vi "RunTimeObjectsSectionUI.vi"() -> ()   [LabVIEW 2015, in "RunTimeObjectsSection.lvclass"]
uses:
  RunTimeObjectsSection.lvclass
  <vilib>/NI/Configuration Framework/Node/NodeRef.ctl
  <vilib>/NI/Configuration Framework/Node/NISE_CEF_Node.lvclass
  <vilib>/NI/AMC/Message Queue.ctl
  <vilib>/NI/AMC/Message.ctl
  <vilib>/NI/Tools/Keyed Array/KeyedArray.ctl
  <vilib>/NI/Configuration Framework/Node/UserEventRef.ctl
  <vilib>/NI/Configuration Framework/Controls/EventCluster.ctl
  <vilib>/Utility/sysdir.llb/System Directory Type.ctl
  Controls/RunTimeObjectTypes.ctl
  RunTimeObjectsSection.lvclass/RunTimeObjectsSection.ctl
  Read RunTimeObjectType.vi
  subVI/Global Settings.vi
  Configuration Tool.lvlib
  <vilib>/NI/Tools/Keyed Array/Tools_KeyedArray.lvlib
  <vilib>/NI/AMC/AMC.lvlib
  <vilib>/NI/Configuration Framework/NISE_CEF_TreeControl.lvlib
panel:
  in  "Main UI Tab":enum32{"Page Group"}(tab)
  in  "WebBrowser":refnum<k7>(container)
  in  "user event":T1
  in  "main queue":T2
  in  "node ref":T3
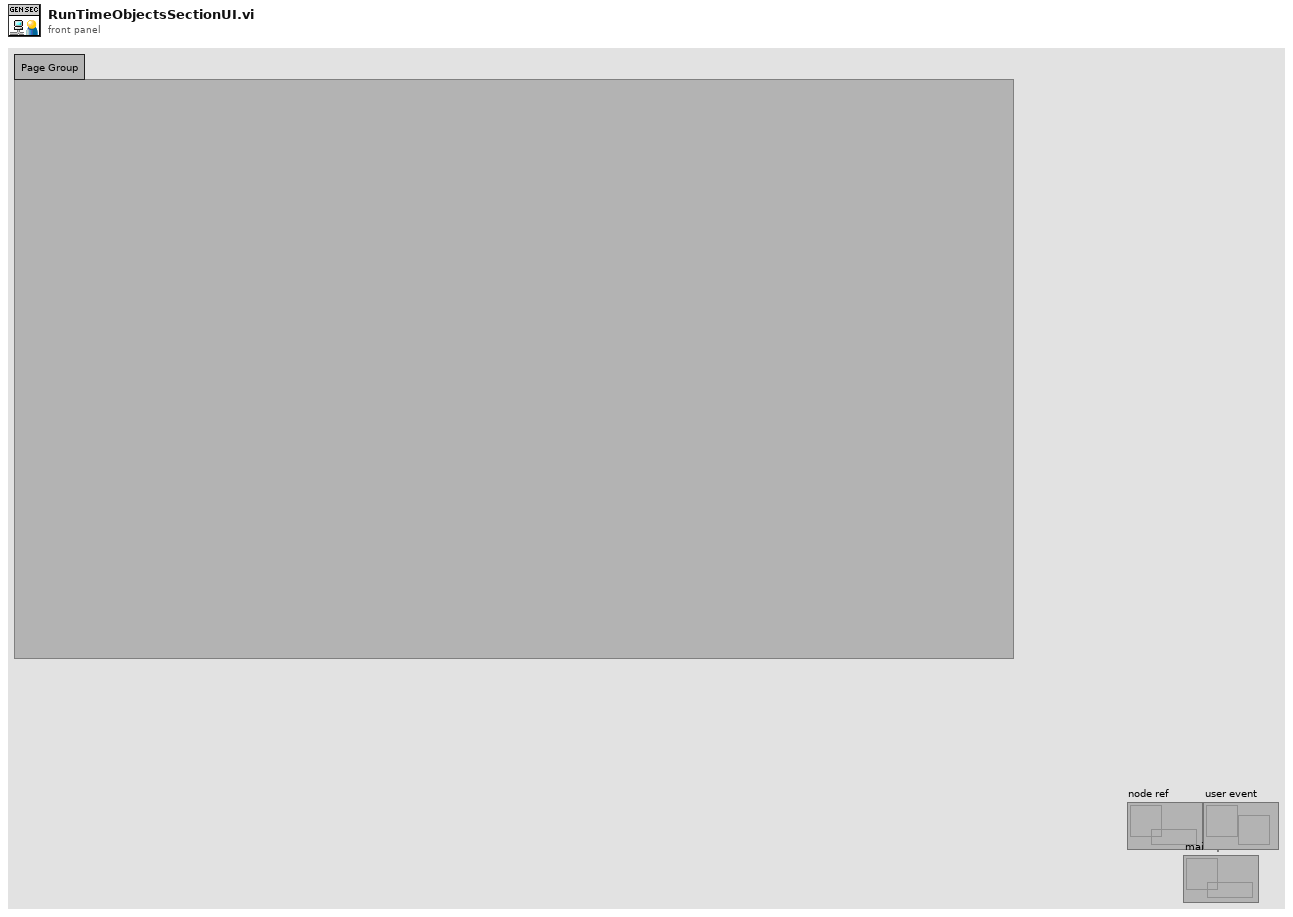
[diagram p1: front panel]
types:
  T1 = typedef "NISE_CEF_Node.lvclass/UserEventRef.ctl" = refnum<user-event>
  T2 = typedef "AMC.lvlib/Message Queue.ctl" = refnum<queue>
  T3 = typedef "NISE_CEF_Node.lvclass/NodeRef.ctl" = refnum<data-value>
  T4 = typedef "Configuration Tool.lvlib/RunTimeObjectTypes.ctl" = enum16{"ActionVIs", "ButtonList", "RunTimeMenu"}
  T5 = typedef "System Directory Type.ctl" = i32
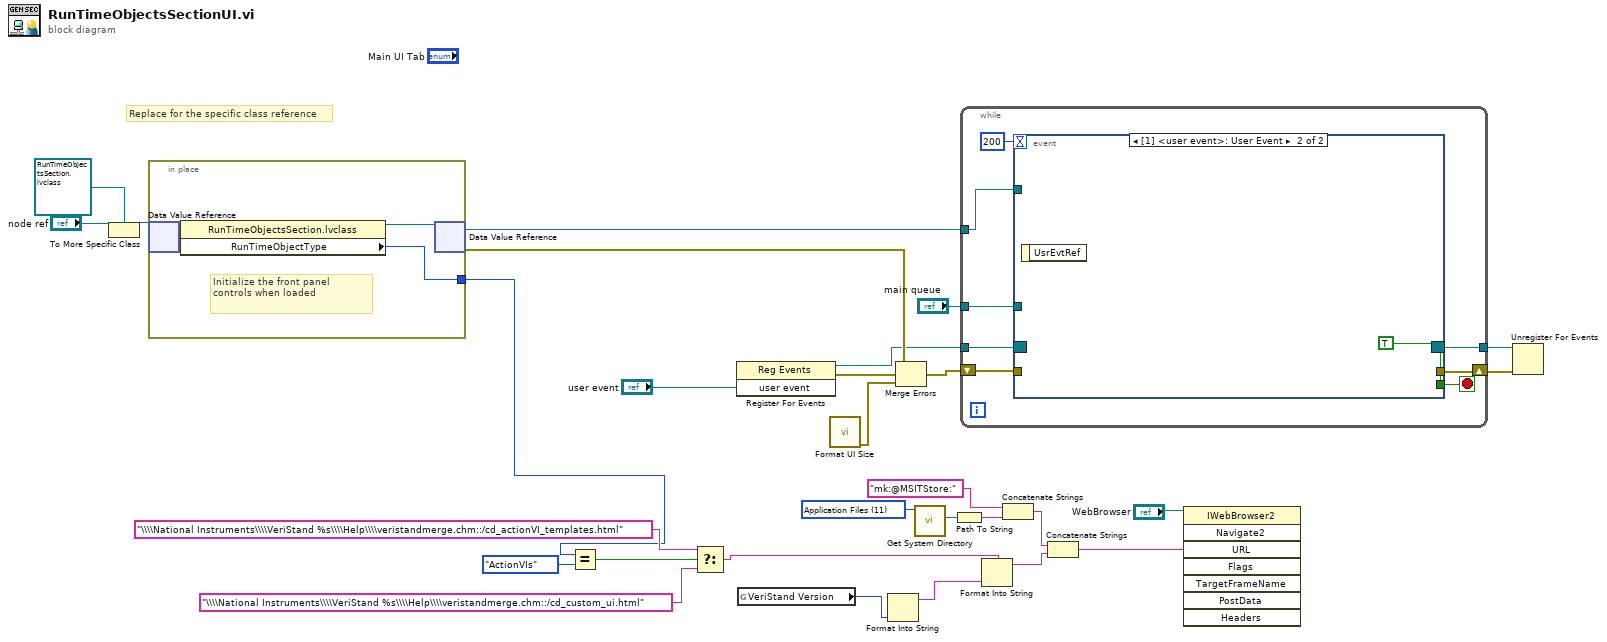
[diagram p0: block diagram]
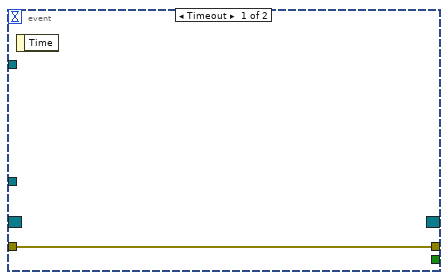
[diagram p2: hidden frame]
diagram:
  w29 = T5 11 items=["User Home"=0, "User Desktop"=1, "User Documents"=2, "User Application Data"=3, "User Preferences"=4, "User Temporary"=5, "Public Documents"=6, "Public Application Data"=7, "Public Preferences"=8, "Public Cache"=13, "System Core Libraries"=9, "System Installed Libraries"=10, "Application Files"=11, "Boot Volume Root"=12] ("system directory type")
  # "Replace for the specific class reference"
  n1 = To More Specific Class(target class=refnum<data-value> refnum ("data value reference"), reference="node ref") -> (specific class reference=w20:refnum<data-value>)  [unwired: 1 in, 1 out]
  n2 = in-place {
    in-place-border: [w30] -> w11
    # "Initialize the front panel controls when loaded"
    n3 = in-place-dvr #1(w20) -> (w32:refnum<class "RunTimeObjectsSection.lvclass">)  [unwired: 1 out]
    n4 = property class="RunTimeObjectsSection.lvclass"(reference=w32) -> (reference out=w31:refnum<class "RunTimeObjectsSection.lvclass">, "RunTimeObjectType"=w30:T4)  [unwired: 1 in, 1 out]
    n5 = in-place-dvr #1(w31) -> (w22:refnum<data-value>, w18:errorcluster)
  }
  n6 = Equal?(x=w11, y=RunTimeObjectTypes."ActionVIs") -> (x = y?=w15:bool)
  n7 = Select(t="\\\\National Instruments\\\\VeriStand %s\\\\Help\\\\veristandmerge.chm::/cd_actionVI_templates.html", s=w15, f="\\\\National Instruments\\\\VeriStand %s\\\\Help\\\\veristandmerge.chm::/cd_custom_ui.html") -> (s? t:f=w13:string)
  n8 = register-events("user event") -> (reference out=w8:refnum<event-registration>, error out=w5:errorcluster)  [unwired: 2 in]
  n9 = global read "Global Settings.vi" "VeriStand Version"() -> (w2:enum16{"2013", "2014", "2015", "2016"})
  n10 = call "Format UI Size.vi"() -> ("error out"=w3:errorcluster)  [unwired: 11 in]
  n11 = Format Into String(w2) -> (resulting string=w1:string)  [unwired: 3 in, 1 out]
  n12 = Merge Errors(w18, w5, w3) -> (w4:errorcluster)
  n13 = call <vilib>:"Get System Directory.vi"("system directory type"=w29) -> ("system directory"=w28:path)  [unwired: 10 in]
  n14 = Path To String(path=w28) -> (string=w27:string)
  n15 = while {
    tunnel: w22 -> [w40]
    tunnel: "main queue" -> [w39]
    tunnel: w8 -> [w37]
    tunnel: [w36] -> w7
    shift-right: [w34] -> w6
    shift-left: w4 -> [w33]
    stop <- w35 stop-if-true
    n16 = event shown="[1] <user event>: User Event" {
      selector: w37 -> [_ _]
      dyn-events: [_ _] -> w36
      timeout: 200 -> [_ _]
      tunnel: w40 -> [_ _]
      tunnel: w39 -> [_ _]
      tunnel: [_ TRUE] -> w35
      tunnel: [w41 _] -> w34
      tunnel: w33 -> [w41 _]
      event Timeout {
        n17 = event-data() -> ()  [unwired: 1 in, 1 out]
      }
      event User Event {
        n18 = event-data() -> ()  [unwired: 1 in, 1 out]
      }
    }
  }
  n19 = Format Into String(format string=w13, w1) -> (resulting string=w24:string)  [unwired: 2 in, 1 out]
  n20 = Concatenate Strings("mk:@MSITStore:" ("concatenated string"), w27) -> (w25:string)
  n21 = Concatenate Strings(w25, w24) -> (w12:string)
  n22 = invoke class="IWebBrowser2" method="Navigate2"(reference="WebBrowser", "URL"=w12) -> ()  [unwired: 6 in, 8 out]
  n23 = Unregister For Events(event registration refnum=w7, error in=w6) -> ()  [unwired: 1 out]
